vi "CAN FlexLogger Test Sender.vi"() -> ()   [LabVIEW 2026]
doc: "Sends known test values on CAN (eDyno_NVH_PoC database) so FlexLogger signal decoding can be checked without the simulator.\n\nEvery 10 ms: DynoSts_SpeedAct ramps 1000 -> 3990 rpm every 3 s, DynoSts_BlockCounter = loop count, DynoSts_Mode = 1, FltSts_ActiveId steps 0..6 every 2 s, FltSts_Freq_1x = speed/60.\n\nStop eDyno NVH Accel Simulator.vi first (both write the same frames on CAN1). Bus settings (CAN FD+BRS, 500k/2M) come from the database alias."
uses:
  <vilib>/xnet/xnet.llb/XNET Create Session (Generic).vi
  <vilib>/xnet/xnet.llb/XNET Write (Signal Single-point).vi
panel:
  out "Values Sent":dbl[](array[numeric])
  out "Loop Count":dbl
  in  "STOP":bool
  in  "XNET Database":string="eDyno_NVH_PoC"
  in  "CAN Interface":string="CAN1"
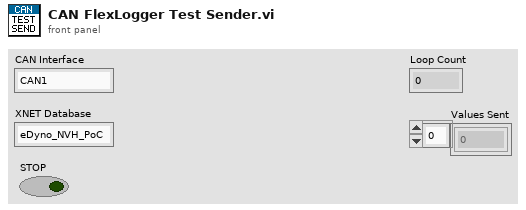
[diagram p1: front panel]
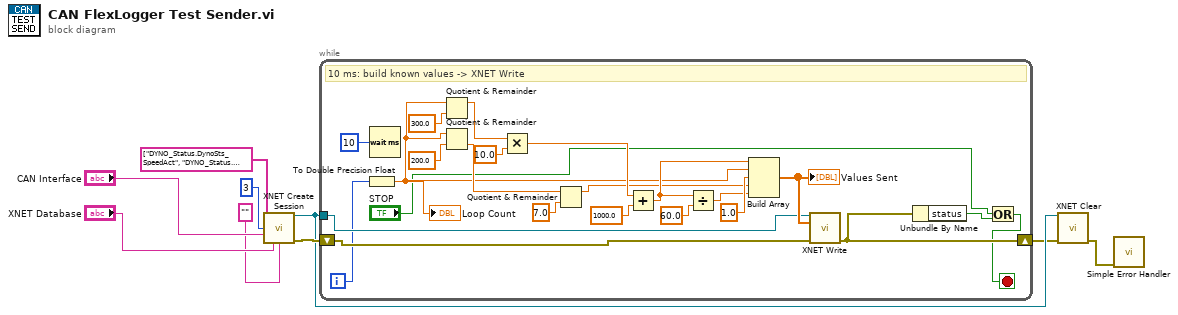
[diagram p0: block diagram]
diagram:
  n1 = call-poly <vilib>:"XNET Create Session.vi"("list (empty)"=string[] ["DYNO_Status.DynoSts_SpeedAct", "DYNO_Status.DynoSts_BlockCounter", "DYNO_Status.DynoSts_Mode", "SIM_FaultStatus.FltSts_ActiveId", "SIM_FaultStatus.FltSts_Freq_1x"] ("signals"), "mode"=u32 3 ("Signal Output Single-point"), "interface"="CAN Interface", "database (:memory:)"="XNET Database", "cluster (empty)"="" ("cluster")) -> ("session out"=w3:refnum<k21>, "error out"=w4:errorcluster)  [unwired: 9 in]
  n2 = while {
    tunnel: w3 -> [w14]
    shift-right: [w13] -> w2
    shift-left: w4 -> [w12]
    i -> [w10]
    stop <- w11 stop-if-true
    # "10 ms: build known values -> XNET Write"
    n3 = To Double Precision Float(number=w10) -> (double precision float=w21:dbl)
    "Loop Count" <- w21
    n4 = Wait (ms)(milliseconds to wait=10 ("10 ms")) -> ()  [unwired: 1 out]
    n5 = Quotient & Remainder(x=w21, y=300.0 ("300")) -> (x-y*floor(x/y)=w30:dbl)  [unwired: 1 out]
    n6 = Quotient & Remainder(x=w21, y=200.0 ("200")) -> (floor(x/y)=w25:dbl)  [unwired: 1 out]
    n7 = Multiply(x=w30, y=10.0 ("10 rpm/step")) -> (x*y=w28:dbl)
    n8 = Quotient & Remainder(x=w25, y=7.0 ("7")) -> (x-y*floor(x/y)=w19:dbl)  [unwired: 1 out]
    n9 = Add(x=w28, y=1000.0 ("1000 rpm")) -> (x+y=w22:dbl)
    n10 = Divide(x=w22, y=60.0 ("60")) -> (x/y=w18:dbl)
    n11 = Build Array(w22, w21, 1.0 ("mode 1"), w19, w18) -> (w17:dbl[])
    "Values Sent" <- w17
    n12 = call-poly <vilib>:"XNET Write.vi"("session in"=w14, "data"=w17, "error in (no error)"=w12) -> ("error out"=w13:errorcluster)  [unwired: 11 in, 1 out]
    n13 = Unbundle By Name(w13) -> ("status"=w15:bool)
    n14 = Or(x="STOP", y=w15) -> (x .or. y?=w11:bool)
  }
  n15 = call <vilib>:"XNET Clear.vi"("session in"=w3, "error in (no error)"=w2) -> ("error out"=w1:errorcluster)  [unwired: 13 in]
  n16 = call <vilib>:"Simple Error Handler.vi"("error in (no error)"=w1) -> ()  [unwired: 4 in, 5 out]
